vi "[ce] CalcExpress - Eval Script.vi"(5 "VC Handle":T3=-1, 6 "error in":errorcluster, 7 "params":T2={"autoVar"=TRUE, "enCpx"=TRUE}, 8 "repeat (1)":i32=1, 9 "CE InstanceRef":T4) -> (0 "error out":errorcluster, 1 "value type":T1=enum."DBL Number", 2 "numeric value":dbl, 3 "dup CE InstanceRef":T4, 4 "dup VC Handle":T3=-1)   [LabVIEW 2021]
doc: "This VI evaluates previously parsed CalcExpress expressions and sequential scripts. To process non-sequential scripts that contain loops and conditional branching, use <b>CSE VIs</b>. Refer to the VI help for more details.\n\n<b>VC Handle</b> specifies the handle of a variable context. CalcExpress accesses variables using this handle. Pass a valid handle to this terminal if the expression uses variables; otherwise, you can leave this input unwired.\n\n<b>expression</b> specifies the CalcExpress expression or sequential script to be executed.\n\n<b>repeat</b> control specifies the number of times an expression is evaluated. The default value is 1.\n\n<b>params</b> cluster specifies optional parameters influencing evaluation:\n <b>autoVar</b> : if it is TRUE (default) and a non-existent variable appears as the left-hand operand in the assignment operator, CalcExpress implicitly creates the variable. If it is FALSE, all variables in the expression must be explicitly created either before or during evaluation.\n <b>enCpx</b> : enables (TRUE, default) or disables (FALSE) the ability to perform operations on operands of data types other than <b>DBL Number</b>.\n\n<b>numeric value</b> returns the numeric value (<b>DBL Number</b>) of the expression.\n\n<b>value type</b> indicates the data type of the expression value.\n\n::: CalcExpress Toolkit :::\nCopyright (c) 2000-2026 Konstantin Shifershteyn. All rights reserved."
uses:
  cetypes.llb/CalcExpress Instance RefNum.ctl
  cetypes.llb/VarMan Variable Context Handle.ctl
  cetypes.llb/CalcExpress Execution Options.ctl
  cetypes.llb/CalcExpress Data Type.ctl
  cersrc/celveng32.dll
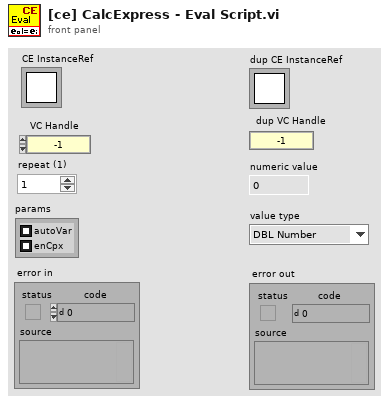
[diagram p1: front panel]
types:
  T1 = typedef "CalcExpress Data Type.ctl" = enum32{"String", "DBL Number", "identifier", "1D Array of DBL", "2D Array of DBL", "CDB Number", "1D Array of CDB", "2D Array of CDB", "1D Array of String", "2D Array of String", "Unknown data type"}
  T2 = typedef "CalcExpress Execution Options.ctl" = cluster{"autoVar":bool, "enCpx":bool}
  T3 = typedef "VarMan Variable Context Handle.ctl" = i32
  T4 = typedef "CalcExpress Instance RefNum.ctl" = refnum<k1>
  T5 = enum32{"String", "DBL Number", "identifier", "1D Array of DBL", "2D Array of DBL", "CDB Number", "1D Array of CDB", "2D Array of CDB", "1D Array of String", "2D Array of String", "Unknown data type"}
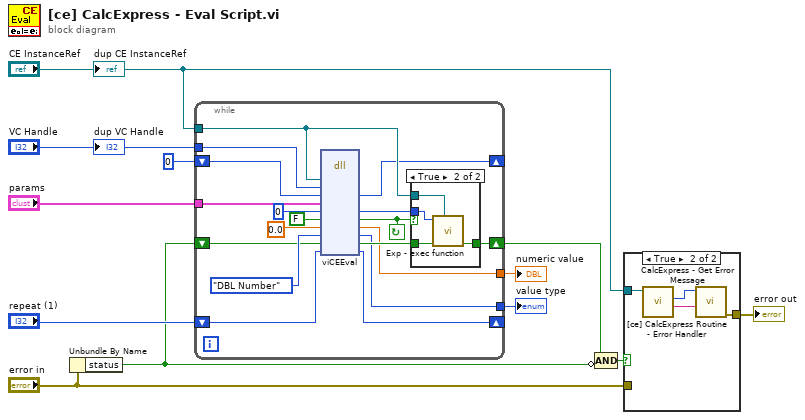
[diagram p0: block diagram]
diagram:
  n1 = Unbundle By Name("error in") -> ("status"=w5:bool)
  n2 = while {
    shift-left: "repeat (1)" -> [w21]
    shift-right: [w20] -> _
    tunnel: [w18] -> w7
    tunnel: [w17] -> w8
    tunnel: "VC Handle" -> [w28]
    tunnel: "CE InstanceRef" -> [w29]
    shift-left: 0 -> [w27]
    shift-right: [w14] -> _
    shift-left: w5 -> [w22]
    shift-right: [w30] -> w9
    tunnel: "params" -> [w13]
    stop <- w16 continue-if-true
    n3 = dll-call lib="C:/LV Projects/CalcExpress 40 LV2021/vi.lib/addons/CalcExpress/cersrc/celveng*.dll" fn="viCEEval"("iRef"=w29, "vch"=w28, "idx"=w27, "cPars"=w13, "opdNum"=0, "NE"=FALSE, "num"=0.0 ("numeric value"), "type"=T5."DBL Number" ("data type"), "erf"=w22, "rept"=w21) -> ("idx"=w14:i32, "opdNum"=w15:i32, "NE"=w16:bool, "num"=w17:dbl, "type"=w18:T5, "erf"=w19:bool, "rept"=w20:i32)  [unwired: 7 in, 2 out]
    n4 = case shown="True" w16 {
      tunnel: [w31 w35] -> w30
      tunnel: w19 -> [w31 w34]
      tunnel: w15 -> [_ w33]
      tunnel: w29 -> [_ w32]
      frame False {
      }
      frame True {
        n5 = call "Exp - exec function.vi"("CE InstanceRef"=w32, "error in"=w34, "ParNum"=w33) -> ("error out"=w35:bool)  [unwired: 6 in]
      }
    }
  }
  "numeric value" <- w8
  "value type" <- w7
  n6 = Compound Arithmetic op=AND(w9, invert w5) -> (w11:bool)
  n7 = case shown="True" w11 {
    tunnel: "error in" -> [w36 _]
    tunnel: [w36 w40] -> w12
    tunnel: "CE InstanceRef" -> [_ w38]
    frame False {
    }
    frame True {
      n8 = call "CalcExpress - Get Error Message.vi"("CE InstanceRef"=w38) -> ("error description"=w39:string, "error code"=w37:i32)  [unwired: 5 in, 2 out]
      n9 = call "[ce] CalcExpress Routine - Error Handler.vi"("error msg"=w39, "error code"=w37) -> ("error out"=w40:errorcluster)  [unwired: 7 in]
    }
  }
  "error out" <- w12
  "dup CE InstanceRef" <- "CE InstanceRef"
  "dup VC Handle" <- "VC Handle"
